vi "Set FPGA Bitfile.vi"(8 "error in":errorcluster, 10 "FPGA bitfile path":path, 11 "FPGA addon refnum in":T1=18446744073709551615 format="%.0x") -> (0 "error out":errorcluster, 3 "FPGA addon refnum out":T1=18446744073709551615 format="%.0x")   [LabVIEW 2020, in "Scripting API.lvlib"]
doc: "Loads and configures the FPGA addon custom device with the FPGA bitfile specified by the \"FPGA bitfile path\" input."
uses:
  Scripting API.lvlib
  <vilib>/NI VeriStand/Custom Device API/Custom Device Item Ref.ctl
  Addon/Addon Shared/Types/FG Action.ctl
  Addon/Addon Shared/SubVIs/Constants.vi
  <vilib>/NI VeriStand/Custom Device API/NI VeriStand - Get Item Property.vi
  <vilib>/NI VeriStand/Custom Device API/Get Item Property (Path).vi
  <vilib>/NI VeriStand/Custom Device API/Get Item Property (String).vi
  <vilib>/NI VeriStand/Custom Device API/Get Item Property (Boolean).vi
  <vilib>/NI VeriStand/Custom Device API/NI VeriStand - Set Item Property.vi
  <vilib>/NI VeriStand/Custom Device API/Set Item Property (Path).vi
  <vilib>/NI VeriStand/Custom Device API/Set Item Property (String).vi
  <vilib>/NI VeriStand/Custom Device API/Set Item Property (Boolean).vi
  Addon/Addon Shared/FPGA Addon Shared.lvlib
  Addon/Addon System Explorer/FPGA Addon System Explorer.lvlib
  <vilib>/NI VeriStand/Custom Device API/Custom Device API.lvlib
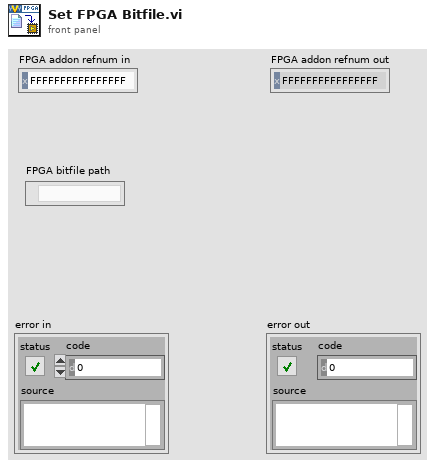
[diagram p1: front panel]
types:
  T1 = typedef "Custom Device API.lvlib/Custom Device Item Ref.ctl" = u64
  T2 = typedef "FPGA Addon Shared.lvlib/FG Action.ctl" = enum8{"GET", "SET"}
  T3 = typedef "FPGA Addon Shared.lvlib/FPGA Settings.ctl" = cluster{"Bitfile path":path, "RIO Device Address":string, "Group":bool}
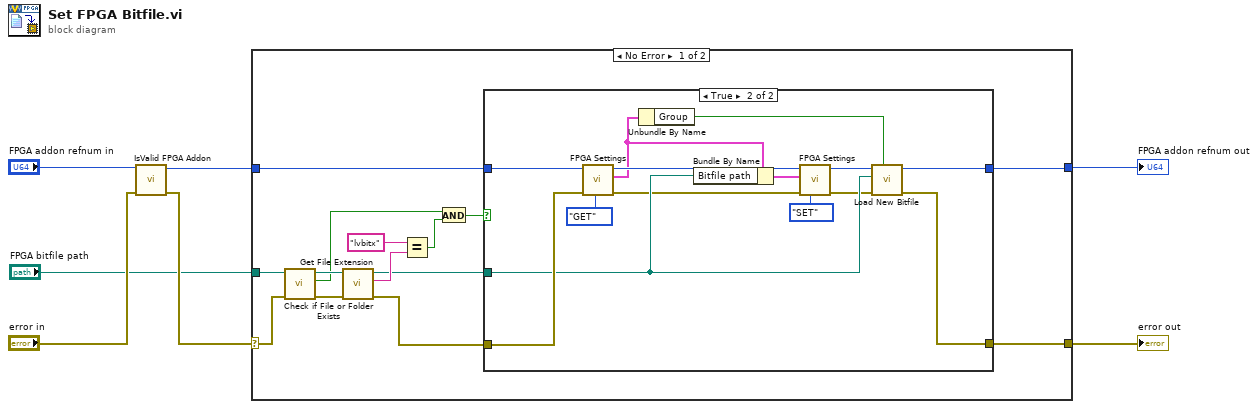
[diagram p0: block diagram]
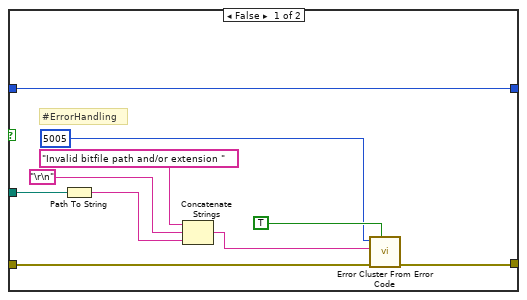
[diagram p2: hidden frame]
diagram:
  n1 = call "IsValid FPGA Addon.vi"("error in"="error in", "FPGA Addon refnum in"="FPGA addon refnum in") -> ("error out"=w6:errorcluster, "FPGA Addon refnum out"=w7:T1)  [unwired: 8 in]
  n2 = case shown="No Error" w6 {
    selector: w6 -> [w11 w46]
    tunnel: w7 -> [w21 w47]
    tunnel: [w19 w46] -> w1
    tunnel: [w20 w47] -> w4
    tunnel: "FPGA bitfile path" -> [w12 _]
    frame No Error {
      n3 = call <vilib>:"Check if File or Folder Exists.vi"("error in (no error)"=w11, "path"=w12) -> ("error out"=w18:errorcluster, "file or folder exists?"=w16:bool, "dup path"=w17:path)  [unwired: 7 in]
      n4 = call <vilib>:"Get File Extension.vi"("error in (no error)"=w18, "file"=w17) -> ("error out"=w10:errorcluster, "lowercase file extension"=w13:string, "dup file"=w8:path)  [unwired: 5 in, 2 out]
      n5 = Equal?(x="lvbitx", y=w13) -> (x = y?=w14:bool)
      n6 = And(x=w16, y=w14) -> (x .and. y?=w9:bool)
      n7 = case shown="True" w9 {
        tunnel: w21 -> [w31 w45]
        tunnel: [w31 w42] -> w20
        tunnel: [w23 w41] -> w19
        tunnel: w10 -> [w24 w40]
        tunnel: w8 -> [w22 w35]
        frame False {
          # "#ErrorHandling"
          n8 = Path To String(path=w22) -> (string=w30:string)
          n9 = Concatenate Strings("Invalid bitfile path and/or extension " ("error message (\"\")"), "\r\n", w30) -> (w29:string)
          n10 = call <vilib>:"Error Cluster From Error Code.vi"("show call chain? (False)"=TRUE, "error in (no error)"=w24, "error message (\"\")"=w29, "error code (0)"=5005) -> ("error out"=w23:errorcluster)  [unwired: 5 in]
        }
        frame True {
          n11 = call "FPGA Settings.vi"("Action"=FG_Action."GET", "error in (no error)"=w40, "Item Ref"=w45) -> ("error out"=w33:errorcluster, "FPGA Settings"=w36:T3, "Item Ref out"=w38:T1)  [unwired: 6 in]
          n12 = Unbundle By Name(w36) -> ("Group"=w43:bool)
          n13 = Bundle By Name(cluster=w36, "Bitfile path"=w35) -> (w34:T3)
          n14 = call "FPGA Settings.vi"("Action"=FG_Action."SET", "error in (no error)"=w33, "FPGA Settings"=w34, "Item Ref"=w38) -> ("error out"=w32:errorcluster, "Item Ref out"=w37:T1)  [unwired: 5 in, 1 out]
          n15 = call "Load New Bitfile.vi"("Group"=w43, "error in (no error)"=w32, "NewVal"=w35, "Item Ref in"=w37) -> ("error out"=w41:errorcluster, "Section Ref out"=w42:T1)  [unwired: 6 in]
        }
      }
    }
    frame Error {
    }
  }
  "error out" <- w1
  "FPGA addon refnum out" <- w4
